vi "FinalDemo.vi"   [LabVIEW 2016]
uses:
  <vilib>/NXT/Block Support/NXT_InputPort.ctl
  <vilib>/NXT/Block Support/NXT_OutputPort.ctl
  <vilib>/NXT/Dual Mode Library/Sensors/EV3_Color_Color.vi
  <vilib>/NXT/Dual Mode Library/Sensors/EV3_Ultrasonic_CM.vi
  <vilib>/NXT/NXTIO Xnodes/NXTIONodeSubVIs/NXTMoveMotors.vi
  <vilib>/NXT/NXTIO Xnodes/NXTIONodeSubVIs/NXTStopMotors.vi
  <vilib>/NXT/NXTIO Xnodes/AddressXNode/NXTIOAddress.xnode
  PMR_081.lvrbt
  <vilib>/NXT/Subs/LVHSConnector.ctl
  <vilib>/NXT/NXTIO Xnodes/NXTIOXNode/NXTIO.xnode
  <vilib>/NXT/LegoClasses/BrickReference/BrickReference.lvclass
types:
  T1 = typedef "NXT_InputPort.ctl" = u32
  T2 = typedef "ColorSensorColors.ctl" = enum16{"No Color", "Black", "Blue", "Green", "Yellow", "Red", "White", "Brown"}
  T3 = typedef "NXT_OutputPort.ctl" = u8
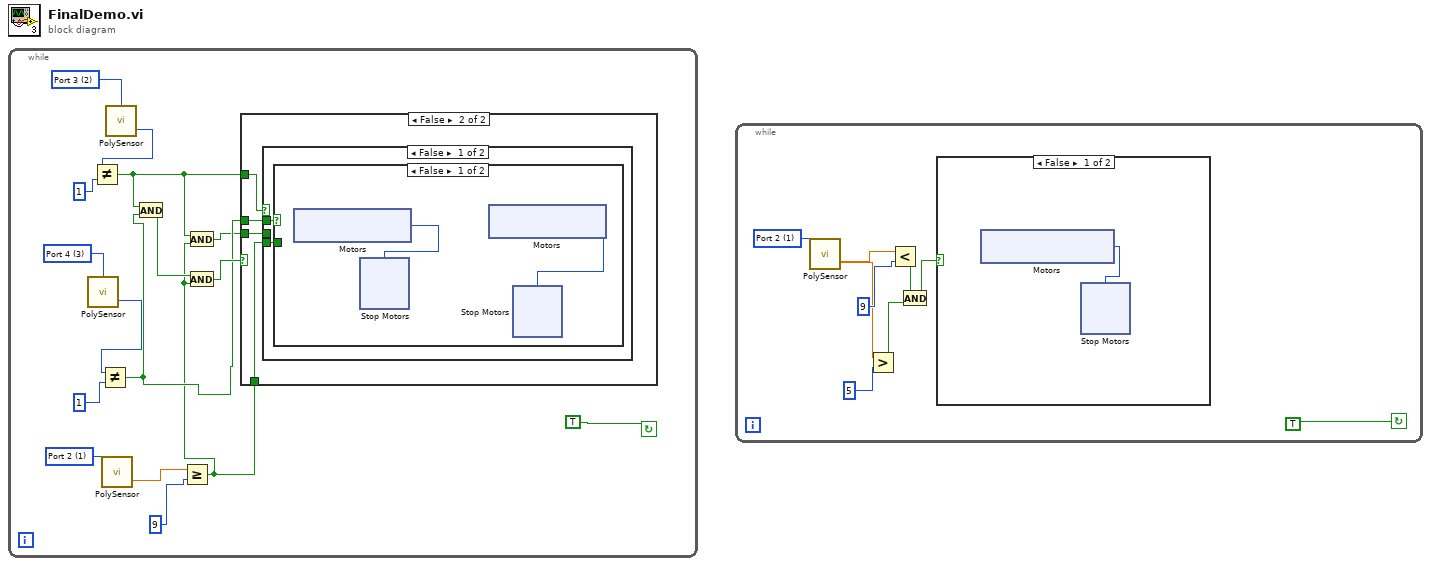
[diagram p0: block diagram]
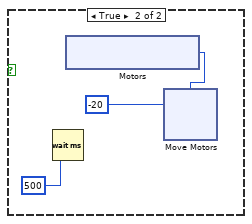
[diagram p2: hidden frame]
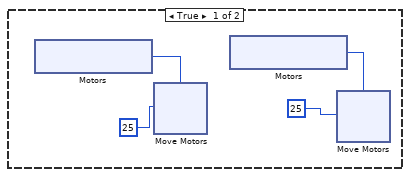
[diagram p3: hidden frame]
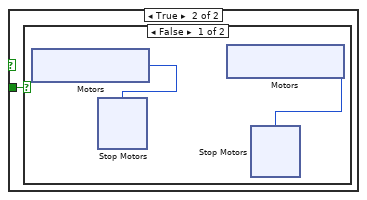
[diagram p4: hidden frame]
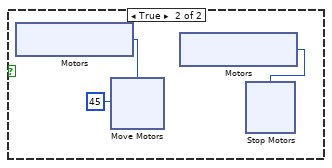
[diagram p5: hidden frame]
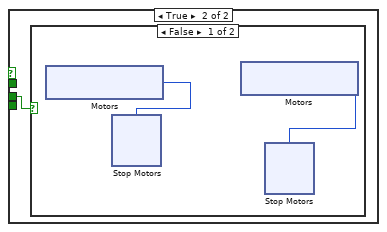
[diagram p6: hidden frame]
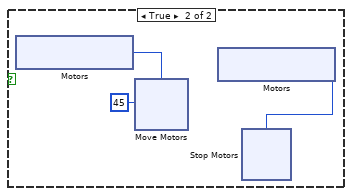
[diagram p7: hidden frame]
diagram:
  n1 = while {
    stop <- TRUE continue-if-true
    w9 = T1 1 items=["Port 1", "Port 2", "Port 3", "Port 4"] ("Port (Port 4)")
    w15 = T1 3 items=["Port 1", "Port 2", "Port 3", "Port 4"] ("Port (Port 1)")
    w16 = T1 2 items=["Port 1", "Port 2", "Port 3", "Port 4"] ("Port (Port 1)")
    n2 = call-poly <vilib>:"PolySensor.vi"("Port (Port 1)"=w15) -> ("Detected Color"=w11:T2)  [unwired: 2 in, 1 out]
    n3 = Not Equal?(x=w11, y=1) -> (x != y?=w4:bool)
    n4 = call-poly <vilib>:"PolySensor.vi"("Port (Port 1)"=w9) -> ("Centimeters"=w5:sgl)  [unwired: 2 in, 1 out]
    n5 = call-poly <vilib>:"PolySensor.vi"("Port (Port 1)"=w16) -> ("Detected Color"=w13:T2)  [unwired: 2 in, 1 out]
    n6 = Not Equal?(x=w13, y=1) -> (x != y?=w2:bool)
    n7 = And(x=w2, y=w4) -> (x .and. y?=w8:bool)
    n8 = Greater Or Equal?(x=w5, y=i16 9 ("Distance (cm)")) -> (x >= y?=w1:bool)
    n9 = And(x=w2, y=w1) -> (x .and. y?=w3:bool)
    n10 = And(x=w8, y=w1) -> (x .and. y?=w7:bool)
    n11 = case shown="False" w7 {
      tunnel: w2 -> [_ w40]
      tunnel: w4 -> [_ w39]
      tunnel: w1 -> [_ w38]
      tunnel: w3 -> [_ w37]
      frame True {
        n12 = xnode "Motors"() -> ("Motor"=w18:T3)
        n13 = xnode "Move Motors"("Power/Speed 1"=i8 25, "Motors"=w18) -> ()  [unwired: 1 in, 1 out]
        n14 = xnode "Motors"() -> ("Motor"=w17:T3)
        n15 = xnode "Move Motors"("Power/Speed 1"=i8 25, "Motors"=w17) -> ()  [unwired: 1 in, 1 out]
      }
      frame False {
        n16 = case shown="False" w40 {
          tunnel: w39 -> [w42 _]
          tunnel: w38 -> [w41 _]
          tunnel: w37 -> [_ w89]
          frame False {
            n17 = case shown="False" w42 {
              tunnel: w41 -> [_ w57]
              frame False {
                n18 = xnode "Motors"() -> ("Motor"=w43:T3)
                n19 = xnode "Stop Motors"("Motors"=w43) -> ()  [unwired: 1 in, 1 out]
                n20 = xnode "Motors"() -> ("Motor"=w44:T3)
                n21 = xnode "Stop Motors"("Motors"=w44) -> ()  [unwired: 1 in, 1 out]
              }
              frame True {
                n22 = case shown="False" w57 {
                  frame False {
                    n23 = xnode "Motors"() -> ("Motor"=w59:T3)
                    n24 = xnode "Stop Motors"("Motors"=w59) -> ()  [unwired: 1 in, 1 out]
                    n25 = xnode "Motors"() -> ("Motor"=w58:T3)
                    n26 = xnode "Stop Motors"("Motors"=w58) -> ()  [unwired: 1 in, 1 out]
                  }
                  frame True {
                    n27 = xnode "Motors"() -> ("Motor"=w73:T3)
                    n28 = xnode "Move Motors"("Power/Speed 1"=i8 45, "Motors"=w73) -> ()  [unwired: 1 in, 1 out]
                    n29 = xnode "Motors"() -> ("Motor"=w72:T3)
                    n30 = xnode "Stop Motors"("Motors"=w72) -> ()  [unwired: 1 in, 1 out]
                  }
                }
              }
            }
          }
          frame True {
            n31 = case shown="False" w89 {
              frame False {
                n32 = xnode "Motors"() -> ("Motor"=w91:T3)
                n33 = xnode "Stop Motors"("Motors"=w91) -> ()  [unwired: 1 in, 1 out]
                n34 = xnode "Motors"() -> ("Motor"=w90:T3)
                n35 = xnode "Stop Motors"("Motors"=w90) -> ()  [unwired: 1 in, 1 out]
              }
              frame True {
                n36 = xnode "Motors"() -> ("Motor"=w105:T3)
                n37 = xnode "Move Motors"("Power/Speed 1"=i8 45, "Motors"=w105) -> ()  [unwired: 1 in, 1 out]
                n38 = xnode "Motors"() -> ("Motor"=w104:T3)
                n39 = xnode "Stop Motors"("Motors"=w104) -> ()  [unwired: 1 in, 1 out]
              }
            }
          }
        }
      }
    }
  }
  n40 = while {
    stop <- TRUE continue-if-true
    w127 = T1 1 items=["Port 1", "Port 2", "Port 3", "Port 4"] ("Port (Port 4)")
    n41 = call-poly <vilib>:"PolySensor.vi"("Port (Port 1)"=w127) -> ("Centimeters"=w124:sgl)  [unwired: 2 in, 1 out]
    n42 = Greater?(x=w124, y=i16 5 ("Distance (cm)")) -> (0:w123:bool)
    n43 = Less?(x=w124, y=i16 9 ("Distance (cm)")) -> (x < y?=w122:bool)
    n44 = And(x=w122, y=w123) -> (x .and. y?=w121:bool)
    n45 = case shown="False" w121 {
      frame False {
        n46 = xnode "Motors"() -> ("Motor"=w129:T3)
        n47 = xnode "Stop Motors"("Motors"=w129) -> ()  [unwired: 1 in, 1 out]
      }
      frame True {
        n48 = Wait (ms)(milliseconds to wait=500) -> ()  [unwired: 1 out]
        n49 = xnode "Motors"() -> ("Motor"=w138:T3)
        n50 = xnode "Move Motors"("Power/Speed 1"=-20, "Motors"=w138) -> ()  [unwired: 1 in, 1 out]
      }
    }
  }
